vi "BT Example 8 - Notifier Synch.vi"() -> ()   [LabVIEW 2021]
uses:
  System/bt_System.lvclass
  BT.lvlib
  Support/Nodes/Composites/abs_Parallel/Support/Status Calculation.ctl
  Support/Nodes/Composites/abs_Parallel/bt_Parallel.lvclass
  Support/Nodes/Decorators/Repeater/Support/Finish On - Type.ctl
  Support/Nodes/Decorators/Repeater/bt_Repeater.lvclass
  Blackboard/Blackboard.lvclass
  Blackboard/Get Value Type/Get I32.vi
  <vilib>/TSA/Abstract Data Classes/Abs_Types/I32 Integer/Abs_I32 Integer.lvclass
  C:/Program Files (x86)/National Instruments/LabVIEW 2021/vi.lib/TSA/Abstract Data Classes/Abs_Types/Integer/Abs_Integer.lvclass
  C:/Program Files (x86)/National Instruments/LabVIEW 2021/vi.lib/TSA/Abstract Data Classes/Abs_Types/Numeric/Abs_Numeric.lvclass
  C:/Program Files (x86)/National Instruments/LabVIEW 2021/vi.lib/TSA/Abstract Data Classes/Abs_Types/Value/Abs_Value.lvclass
  C:/Program Files (x86)/National Instruments/LabVIEW 2021/vi.lib/TSA/Abstract Data Classes/Abs_Types/Type/Abs_Type.lvclass
  C:/Program Files (x86)/National Instruments/LabVIEW 2021/vi.lib/TSA/Abstract Data Classes/Abs_Types/I32 Integer/Abs_I32 Integer.lvclass
  <vilib>/TSA/Abstract Data Classes/Constants/Support/Str/Str.vi
  <vilib>/TSA/Abstract Data Classes/Constants/Support/Str/Const_Str.lvclass
  <vilib>/TSA/Event Log/abs_EventLog/Support/Facility Code.ctl
  <vilib>/TSA/Event Log/abs_EventLog/abs_EventLog.lvclass
  <vilib>/TSA/Event Log/abs_EventLog/Support/Severity Code.ctl
  <vilib>/TSA/Event Log/Event_TextLog/Event_TextLog.lvclass
  <vilib>/TSA/Abstract Data Classes/Abs_Types/I32 Integer/Static Read.vi
  <vilib>/TSA/Abstract Data Classes/Functions/Math/Support/Increment/I32/Method.vi
  <vilib>/TSA/Abstract Data Classes/Functions/Math/Support/Increment/I32/Increment_I32.lvclass
  <vilib>/TSA/Abstract Data Classes/Constants/Support/I32/I32.vi
  <vilib>/TSA/Abstract Data Classes/Constants/Support/I32/Const_I32.lvclass
  <vilib>/TSA/Abstract Data Classes/Functions/Compare/Support/Greater Equal/I32/Method.vi
  <vilib>/TSA/Abstract Data Classes/Functions/Compare/Support/Greater Equal/I32/Greater Equal_I32.lvclass
  C:/Program Files (x86)/National Instruments/LabVIEW 2021/vi.lib/TSA/Event Log/abs_EventLog/abs_EventLog.lvclass
  C:/Program Files (x86)/National Instruments/LabVIEW 2021/vi.lib/TSA/Event Log/Event_TextLog/Event_TextLog.lvclass
  Support/Poly/Log/Log_StringClass.vi
  Support/Nodes/Leaves/Log/bt_Log.lvclass
  C:/Users/timst/Documents/Repositories/LV_Behaviour_Tree/Source/Support/Nodes/Leaves/Leaf/bt_Leaf.lvclass
  C:/Users/timst/Documents/Repositories/LV_Behaviour_Tree/Source/Support/Nodes/abs_Node/bt_Node.lvclass
  C:/Users/timst/Documents/Repositories/LV_Behaviour_Tree/Source/Support/Nodes/Leaves/Log/bt_Log.lvclass
  Support/Nodes/abs_Node/Status.ctl
  Support/Nodes/abs_Node/bt_Node.lvclass
panel:
  out "Event Log":string
  out "Tags Table":string[][](table)
  out "Values":u32[](array[numeric])
  out "error out":errorcluster
  in  "stop":bool
  out "Status":T1
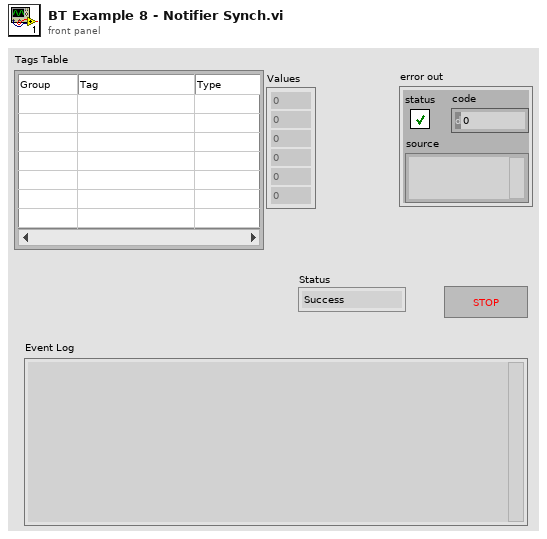
[diagram p1: front panel]
types:
  T1 = typedef "BT.lvlib/bt_Node.lvclass/Status.ctl" = enum16{"Success", "Failure", "Running"}
  T2 = typedef "abs_EventLog.lvclass/Severity Code.ctl" = enum16{"emergency", "alert", "critical", "error", "warning", "notice", "info", "debug"}
  T3 = typedef "abs_EventLog.lvclass/Facility Code.ctl" = enum16{"kernel", "user", "mail", "system daemons", "security/authorization", "syslogd", "line printer", "network news", "uucp", "clock daemon", "security/authorization (alternate)", "FTP daemon", "NTP subsystem", "log audit", "log alert", "clock daemon (alternate)", "local use 0", "local use 1", "local use 2", "local use 3", "local use 4", "local use 5", "local use 6", "local use 7"}
  T4 = typedef "BT.lvlib/bt_Repeater.lvclass/Finish On - Type.ctl" = enum16{"Success", "Failure", "Never"}
  T5 = typedef "BT.lvlib/bt_Parallel.lvclass/Status Calculation.ctl" = enum16{"Succeed on All Succeed", "Failure on All Failure", "Succeed on Any Succeed", "Failure on Any Failure"}
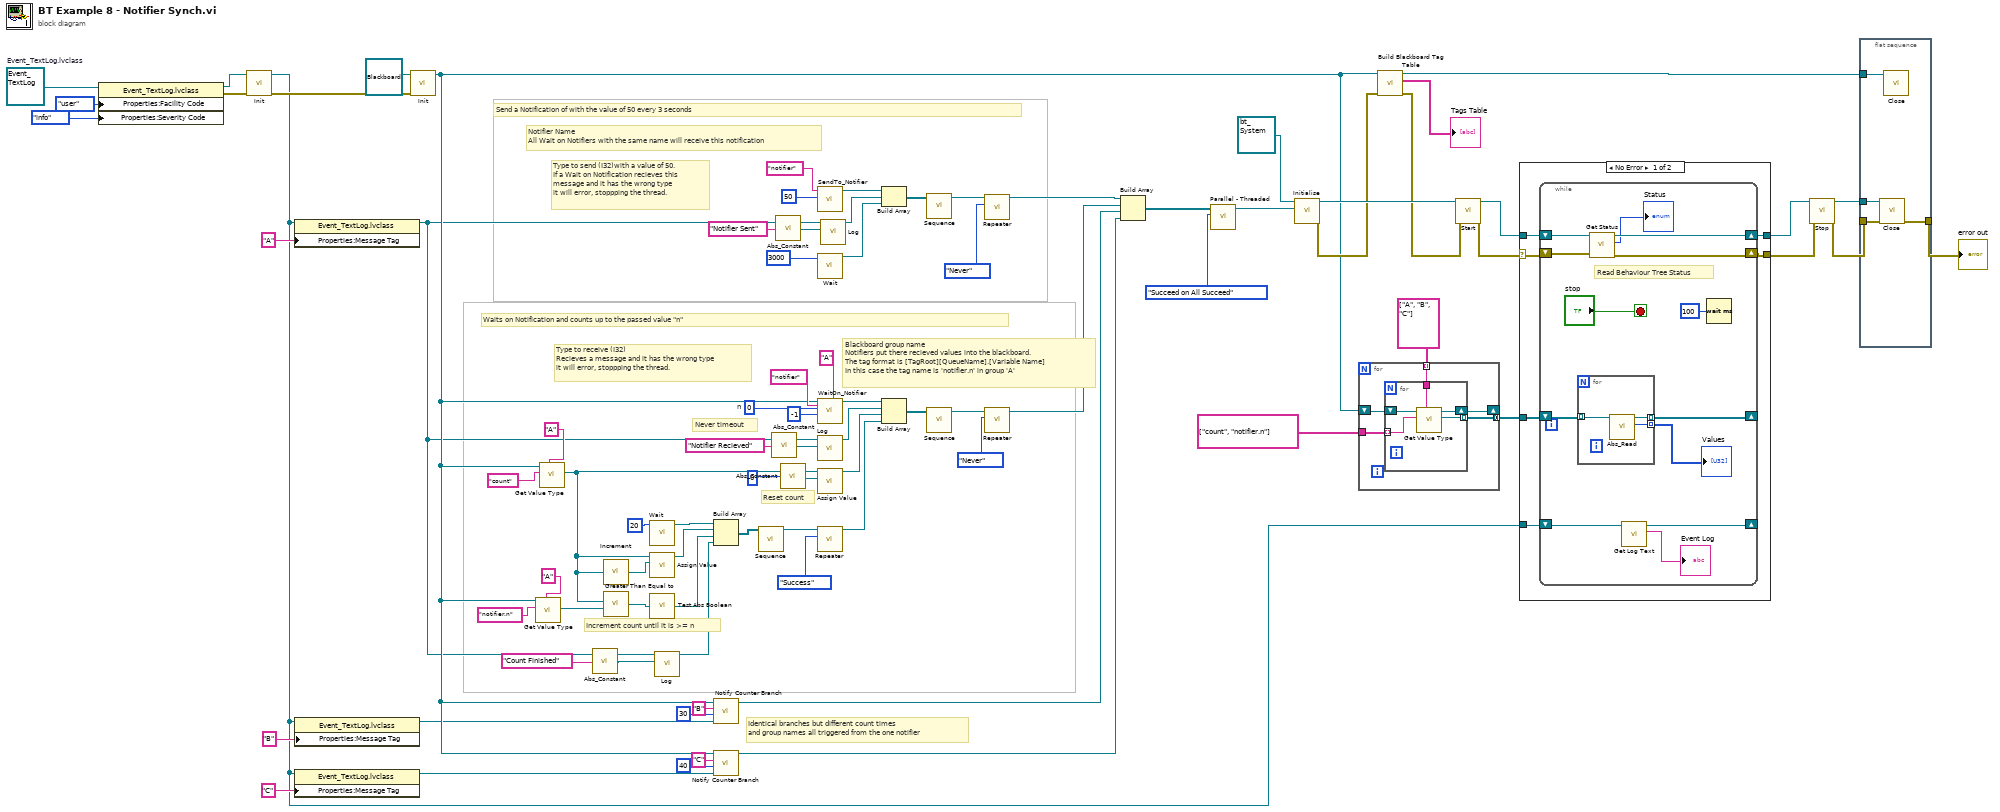
[diagram p0: block diagram]
diagram:
  w11 = refnum<class "Event_TextLog.lvclass"> refnum  # Event_TextLog.lvclass
  w40 = 0  # n
  # "Waits on Notification and counts up to the passed value \"n\""
  # "Increment count until it is >= n"
  # "Reset count"
  # "Identical branches but different count times\nand group names all triggered from the one notifier"
  # "Blackboard group name\nNotifiers put there recieved values into the blackboard.\nThe tag format is [TagRoot][QueueName].[Variable Name]\nIn this case the tag name is 'notifier.n' in group 'A'"
  # "Never timeout"
  # "Type to receive (I32)\nRecieves a message and it has the wrong type\nit will error, stoppping the thread."
  # "Notifier Name\nAll Wait on Notifiers with the same name will receive this notification"
  # "Type to send (I32)with a value of 50.\nIf a Wait on Notification recieves this\nmessage and it has the wrong type\nit will error, stoppping the thread."
  # "Send a Notification of with the value of 50 every 3 seconds"
  n1 = property class="Event_TextLog.lvclass"(reference=w11, "Properties:Facility Code"=Facility_Code."user" ("Facility Code"), "Properties:Severity Code"=Severity_Code."info" ("Severity Code")) -> (reference out=w9:refnum<class "Event_TextLog.lvclass">, error out=w10:errorcluster)  [unwired: 1 in]
  n2 = call-dynamic "Init.vi"("error in (no error)"=w10, "Event_TextLog in"=w9) -> ("error out"=w8:errorcluster, "Event_TextLog out"=w1:refnum<class "Event_TextLog.lvclass">)  [unwired: 8 in]
  n3 = property class="Event_TextLog.lvclass"(reference=w1, "Properties:Message Tag"="A" ("Message Tag")) -> (reference out=w6:refnum<class "Event_TextLog.lvclass">)  [unwired: 1 in, 1 out]
  n4 = property class="Event_TextLog.lvclass"(reference=w1, "Properties:Message Tag"="C" ("Message Tag")) -> (reference out=w2:refnum<class "Event_TextLog.lvclass">)  [unwired: 1 in, 1 out]
  n5 = property class="Event_TextLog.lvclass"(reference=w1, "Properties:Message Tag"="B" ("Message Tag")) -> (reference out=w4:refnum<class "Event_TextLog.lvclass">)  [unwired: 1 in, 1 out]
  n6 = call-dynamic "Init.vi"("error in (no error)"=w8, "bt_Blackboard in"=refnum<class "Blackboard.lvclass"> refnum) -> ("bt_Blackboard out"=w25:refnum<class "Blackboard.lvclass">)  [unwired: 8 in, 1 out]
  n7 = call-poly "Get Value Type.vi"("Tag Group"="A" ("Blackboard Group"), "Tag"="notifier.n", "Blackboard in"=w25) -> ("Value"=w33:refnum<class "Abs_I32 Integer.lvclass">)  [unwired: 5 in, 3 out]
  n8 = call-poly "Get Value Type.vi"("Tag Group"="A" ("Blackboard Group"), "Tag"="count", "Blackboard in"=w25) -> ("Value"=w34:refnum<class "Abs_I32 Integer.lvclass">)  [unwired: 5 in, 3 out]
  n9 = call-poly <vilib>:"Abs_Constant.vi"("String"="Count Finished") -> ("Abs_String.lvclass"=w15:refnum<class "Abs_String.lvclass">)  [unwired: 4 in]
  n10 = call-poly <vilib>:"Increment.vi"("Value"=w34) -> ("Result"=w57:refnum<class "Abs_I32 Integer.lvclass">)  [unwired: 4 in]
  n11 = call-poly <vilib>:"Greater Than Equal to.vi"("Value B"=w33, "Value A"=w34) -> ("Result"=w55:refnum<class "Abs_Boolean.lvclass">)  [unwired: 4 in]
  n12 = call "Wait.vi"("Time (ms)"=u32 20) -> ("Node Out"=w52:refnum<class "bt_Node.lvclass">)  [unwired: 10 in]
  n13 = call "Assign Value.vi"("Assigned Value"=w57, "Value"=w34) -> ("Node Out"=w56:refnum<class "bt_Node.lvclass">)  [unwired: 9 in]
  n14 = call "Test Abs Boolean.vi"("Abs_Boolean.lvclass"=w55) -> ("abs_Node"=w54:refnum<class "bt_Node.lvclass">)  [unwired: 4 in]
  n15 = call-poly "Log.vi"("Message"=w15, "EventLog"=w6) -> ("node out"=w14:refnum<class "bt_Log.lvclass">)  [unwired: 9 in]
  n16 = Build Array(w52, w56, w54, w14) -> (w62:refnum<class "bt_Node.lvclass">[])
  n17 = call "Notify Counter Branch.vi"("EventLog"=w4, "Time (ms)"=u32 30, "Blackboard Group"="B", "Blackboard in"=w25) -> ("bt_Node out"=w35:refnum<class "bt_Node.lvclass">)  [unwired: 7 in]
  n18 = call "Notify Counter Branch.vi"("EventLog"=w2, "Time (ms)"=u32 40, "Blackboard Group"="C", "Blackboard in"=w25) -> ("bt_Node out"=w24:refnum<class "bt_Node.lvclass">)  [unwired: 7 in]
  n19 = call "Sequence.vi"("Nodes"=w62) -> ("Node"=w63:refnum<class "bt_Node.lvclass">)  [unwired: 10 in]
  n20 = call-poly <vilib>:"Abs_Constant.vi"("String"="Notifier Recieved") -> ("Abs_String.lvclass"=w18:refnum<class "Abs_String.lvclass">)  [unwired: 4 in]
  n21 = call-poly <vilib>:"Abs_Constant.vi"("String"="Notifier Sent") -> ("Abs_String.lvclass"=w21:refnum<class "Abs_String.lvclass">)  [unwired: 4 in]
  n22 = call-poly <vilib>:"Abs_Constant.vi"("Value"=0 ("n")) -> ("Constant"=w58:refnum<class "Abs_I32 Integer.lvclass">)  [unwired: 4 in]
  n23 = call "WaitOn_Notifier.vi"("Blackboard Group"="A", "Notifier Name"="notifier" ("Name"), "Timeout (ms)"=-1, "Message Type"=w40, "bt_Blackboard in"=w25) -> ("Node Out"=w39:refnum<class "bt_Node.lvclass">)  [unwired: 5 in, 1 out]
  n24 = call-poly "Log.vi"("Message"=w18, "EventLog"=w6) -> ("node out"=w17:refnum<class "bt_Log.lvclass">)  [unwired: 9 in]
  n25 = call "Assign Value.vi"("Assigned Value"=w58, "Value"=w34) -> ("Node Out"=w53:refnum<class "bt_Node.lvclass">)  [unwired: 9 in]
  n26 = call "Repeater.vi"("Finish On"=Finish_On_-_Type."Success", "Node In"=w63) -> ("Node Out"=w64:refnum<class "bt_Node.lvclass">)  [unwired: 9 in]
  n27 = call "SendTo_Notifier.vi"("Message"=50, "Queue Name"="notifier" ("Name")) -> ("Node Out"=w78:refnum<class "bt_Node.lvclass">)  [unwired: 9 in]
  n28 = call "Wait.vi"("Time (ms)"=u32 3000) -> ("Node Out"=w75:refnum<class "bt_Node.lvclass">)  [unwired: 10 in]
  n29 = call-poly "Log.vi"("Message"=w21, "EventLog"=w6) -> ("node out"=w22:refnum<class "bt_Log.lvclass">)  [unwired: 9 in]
  n30 = Build Array(w78, w22, w75) -> (w77:refnum<class "bt_Node.lvclass">[])
  n31 = Build Array(w39, w17, w53, w64) -> (w66:refnum<class "bt_Node.lvclass">[])
  n32 = call "Sequence.vi"("Nodes"=w77) -> ("Node"=w43:refnum<class "bt_Node.lvclass">)  [unwired: 10 in]
  n33 = call "Sequence.vi"("Nodes"=w66) -> ("Node"=w65:refnum<class "bt_Node.lvclass">)  [unwired: 10 in]
  n34 = call "Repeater.vi"("Finish On"=Finish_On_-_Type."Never", "Node In"=w43) -> ("Node Out"=w42:refnum<class "bt_Node.lvclass">)  [unwired: 9 in]
  n35 = call "Repeater.vi"("Finish On"=Finish_On_-_Type."Never", "Node In"=w65) -> ("Node Out"=w73:refnum<class "bt_Node.lvclass">)  [unwired: 9 in]
  n36 = Build Array(w42, w73, w35, w24) -> (w80:refnum<class "bt_Node.lvclass">[])
  n37 = call "Parallel - Threaded.vi"("Status Calculation"=Status_Calculation."Succeed on All Succeed", "Nodes"=w80) -> ("Node"=w79:refnum<class "bt_Node.lvclass">)  [unwired: 9 in]
  n38 = call "Initialise.vi"("Behaviour Tree"=w79, "bt_System in"=refnum<class "bt_System.lvclass"> refnum) -> ("error out"=w45:errorcluster, "bt_System out"=w48:refnum<class "bt_System.lvclass">)  [unwired: 8 in]
  n39 = for {
    shift-right: [w90] -> _
    shift-left: w25 -> [w91]
    tunnel: string[] ["A", "B", "C"] ("Blackboard Group") -> [w89] mode=indexing
    tunnel: [w88] -> w31 mode=concatenating
    tunnel: string[] ["count", "notifier.n"] ("Tag") -> [w87]
    n40 = for {
      shift-right: [w95] -> w90
      shift-left: w91 -> [w96]
      tunnel: w89 -> [w94]
      tunnel: [w93] -> w88 mode=indexing
      tunnel: w87 -> [w92] mode=indexing
      n41 = call-poly "Get Value Type.vi"("Tag Group"=w94, "Tag"=w92, "Blackboard in"=w96) -> ("Value"=w93:refnum<class "Abs_I32 Integer.lvclass">, "Blackboard out"=w95:refnum<class "Blackboard.lvclass">)  [unwired: 5 in, 2 out]
    }
  }
  n42 = call "Build Blackboard Tag Table.vi"("error in (no error)"=w45, "Blackboard in"=w25) -> ("error out"=w47:errorcluster, "Table"=→"Tags Table":string[][], "Blackboard out"=w46:refnum<class "Blackboard.lvclass">)  [unwired: 6 in, 1 out]
  n43 = call "Start.vi"("error in (no error)"=w47, "bt_System in"=w48) -> ("error out"=w69:errorcluster, "bt_System out"=w85:refnum<class "bt_System.lvclass">)  [unwired: 8 in]
  n44 = case shown="No Error" w69 {
    selector: w69 -> [w100 w119]
    tunnel: w85 -> [w102 w120]
    tunnel: [w101 w120] -> w82
    tunnel: [w99 w119] -> w67
    tunnel: w31 -> [w98 _]
    tunnel: w1 -> [w97 _]
    frame No Error {
      n45 = while {
        shift-right: [w113] -> w101
        shift-left: w102 -> [w114]
        shift-right: [w109] -> w99
        shift-left: w100 -> [w110]
        shift-right: [w107] -> _
        shift-left: w98 -> [w106]
        shift-right: [w104] -> _
        shift-left: w97 -> [w105]
        stop <- "stop" stop-if-true
        # "Read Behaviour Tree Status"
        n46 = for {
          tunnel: [w118] -> w108 mode=indexing
          tunnel: [w117] -> w107 mode=indexing
          tunnel: w106 -> [w116] mode=indexing
          n47 = call-poly <vilib>:"Abs_Read.vi"("Abs_I32 Integer in"=w116) -> ("Value"=w118:i32, "Abs_I32 Integer out"=w117:refnum<class "Abs_I32 Integer.lvclass">)  [unwired: 8 in, 1 out]
        }
        "Values" <- w108
        n48 = call "Get Status.vi"("error in (no error)"=w110, "bt_System in"=w114) -> ("error out"=w109:errorcluster, "Status"=→"Status":T1, "bt_System out"=w113:refnum<class "bt_System.lvclass">)  [unwired: 7 in]
        n49 = call <vilib>:"Get Log Text.vi"("Event_TextLog in"=w105) -> ("Log Message"=→"Event Log":string, "Event_TextLog out"=w104:refnum<class "Event_TextLog.lvclass">)  [unwired: 8 in, 1 out]
        n50 = Wait (ms)(milliseconds to wait=u32 100) -> ()  [unwired: 1 out]
      }
    }
    frame Error {
    }
  }
  n51 = call "Stop.vi"("error in (no error)"=w67, "bt_System in"=w82) -> ("error out"=w83:errorcluster, "bt_System out"=w84:refnum<class "bt_System.lvclass">)  [unwired: 8 in]
  n52 = flat-sequence {
    tunnel: w84 -> [w124]
    tunnel: w83 -> [w123]
    tunnel: [w122] -> w68
    tunnel: w46 -> [w121]
    frame #0 {
      n53 = call-dynamic "Close.vi"("error in (no error)"=w123, "bt_System in"=w124) -> ("error out"=w122:errorcluster)  [unwired: 8 in, 1 out]
      n54 = call-dynamic "Close.vi"("bt_Blackboard in"=w121) -> ()  [unwired: 9 in, 2 out]
    }
  }
  "error out" <- w68
